vi "Helper Loop.vi"(8 "error in (no error)":errorcluster, 9 "Message Data":variant, 10 "Message":string, 11 "Helper Loop In":refnum<class "Helper Loop.lvclass">) -> (0 "error out":errorcluster, 3 "Helper Loop Out":refnum<class "Helper Loop.lvclass">)   [LabVIEW 2020, in "Helper Loop.lvclass"]
uses:
  Helper Loop.lvclass
  Process/Process.lvclass
  Process/Process.lvclass/Process.ctl
  Process/Public/Lifecycle/Lifecycle State.ctl
  Error Handler Interface/Error Handler Interface.lvclass
  Broadcast Event Helpers/Execution timer.vi
  Logging/Log Error.vi
  Logging/Log Warning.vi
  <vilib>/Utility/error.llb/Clear Errors.vi
  <vilib>/Utility/error.llb/Error Cluster From Error Code.vi
  Broadcast Event Dequeuers/Dequeue Broadcast Message.vi
  Logging/Logging.lvclass
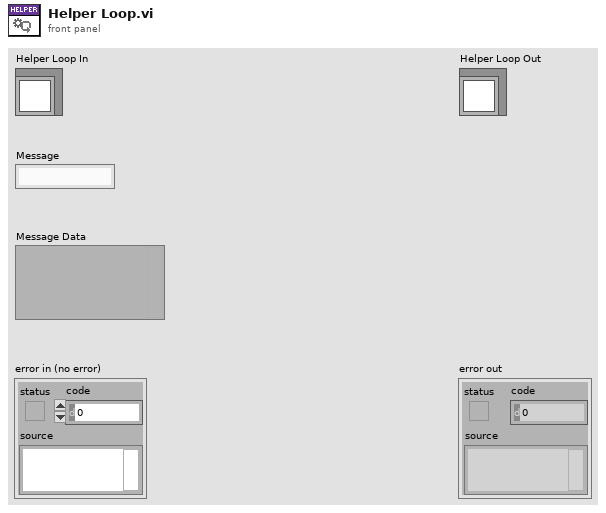
[diagram p1: front panel]
types:
  T1 = typedef "Process.lvclass/Lifecycle State.ctl" = enum16{"Uninitialized", "Initialized", "Started", "Running", "Stopped", "Finished"}
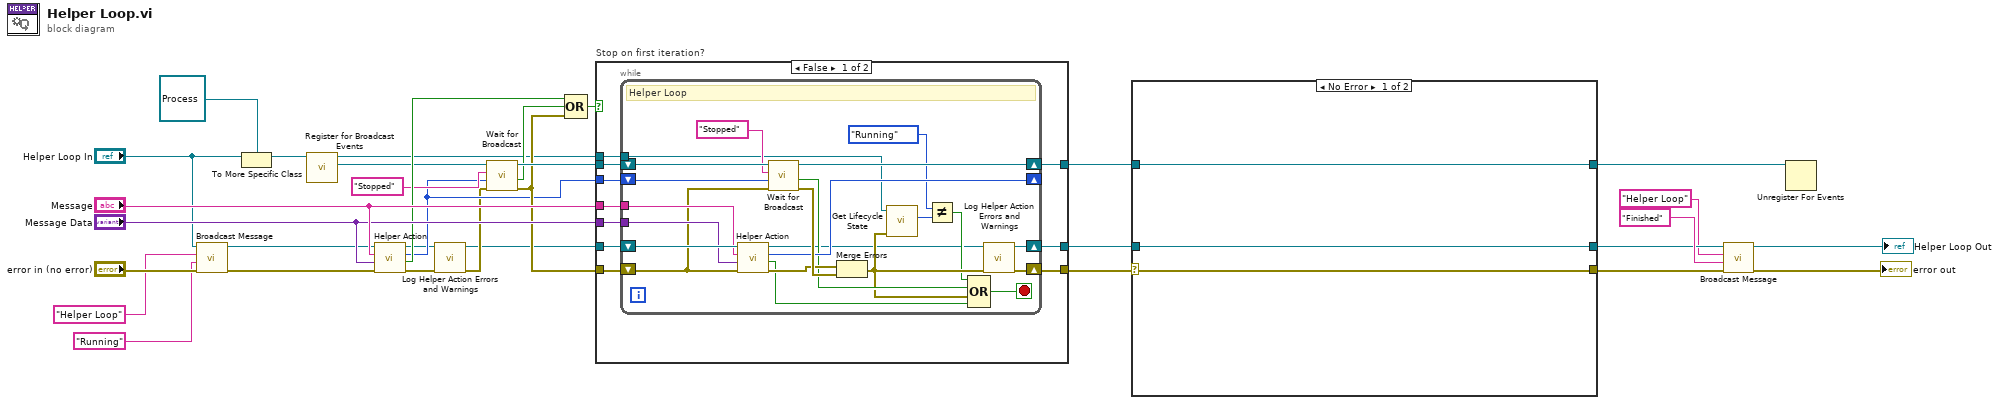
[diagram p0: block diagram]
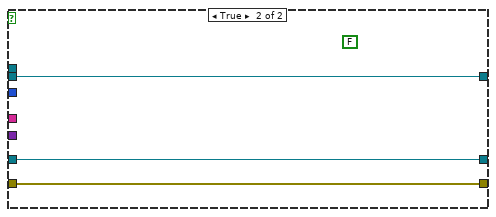
[diagram p2: hidden frame]
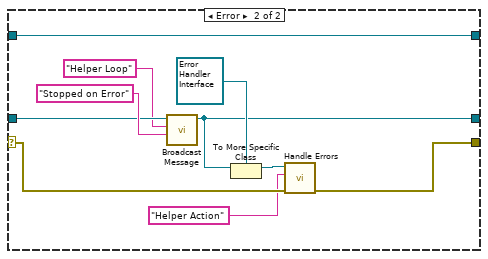
[diagram p3: hidden frame]
diagram:
  n1 = call-dynamic "Broadcast Message.vi"("error in (no error)"="error in (no error)", "Message Data"="Running" ("Message"), "Message"="Helper Loop", "Helper Loop in"="Helper Loop In") -> ("error out"=w8:errorcluster, "Helper Loop out"=w23:refnum<class "Helper Loop.lvclass">)  [unwired: 6 in]
  n2 = To More Specific Class(target class=refnum<class "Process.lvclass"> refnum ("Process.lvclass"), reference="Helper Loop In") -> (specific class reference=w10:refnum<class "Process.lvclass">)  [unwired: 1 in, 1 out]
  n3 = call "Register for Broadcast Events.vi"("Process In"=w10) -> ("Event Registration Refnum Out"=w9:refnum<event-registration>, "Process Out"=w1:refnum<class "Process.lvclass">)  [unwired: 8 in, 1 out]
  n4 = call-dynamic "Helper Action.vi"("error in (no error)"=w8, "Message Data"="Message Data", "Message"="Message", "Helper Loop In"=w23) -> ("error out"=w5:errorcluster, "Exit?"=w24:bool, "Loop Period [ms]"=w6:u32, "Helper Loop Out"=w3:refnum<class "Helper Loop.lvclass">)  [unwired: 4 in]
  n5 = call "Log Helper Action Errors and Warnings.vi"("error in (no error)"=w5, "Helper Loop in"=w3) -> ("error out"=w4:errorcluster, "Helper Loop Out"=w2:refnum<class "Helper Loop.lvclass">)  [unwired: 8 in]
  n6 = call "Wait for Broadcast.vi"("error in (no error)"=w4, "Timeout [ms]"=w6, "Broadcast Message"="Stopped", "Event Registration Refnum in"=w9) -> ("error out"=w20:errorcluster, "Stop Received?"=w13:bool, "Event Registration Refnum out"=w28:refnum<event-registration>)  [unwired: 5 in]
  n7 = Compound Arithmetic op=OR(w24, w13, w20) -> (w25:bool)
  n8 = case "Stop on first iteration?" shown="False" w25 {
    tunnel: [w43 w67] -> w30
    tunnel: [w42 w66] -> w29
    tunnel: [w41 w68] -> w22
    tunnel: w2 -> [w40 w67]
    tunnel: w28 -> [w39 w68]
    tunnel: w20 -> [w38 w66]
    tunnel: "Message" -> [w37 _]
    tunnel: "Message Data" -> [w36 _]
    tunnel: w6 -> [w35 _]
    tunnel: w1 -> [w34 _]
    frame False {
      n9 = while {
        shift-right: [w50] -> w43
        shift-left: w40 -> [w65]
        shift-right: [w51] -> w42
        shift-left: w38 -> [w55]
        tunnel: w37 -> [w62]
        tunnel: w36 -> [w61]
        shift-right: [w57] -> _
        shift-left: w35 -> [w59]
        shift-right: [w56] -> w41
        shift-left: w39 -> [w60]
        tunnel: w34 -> [w49]
        stop <- w64 stop-if-true
        # "Helper Loop"
        n10 = call-dynamic "Helper Action.vi"("error in (no error)"=w55, "Message Data"=w61, "Message"=w62, "Helper Loop In"=w65) -> ("error out"=w58:errorcluster, "Exit?"=w54:bool, "Loop Period [ms]"=w57:u32, "Helper Loop Out"=w44:refnum<class "Helper Loop.lvclass">)  [unwired: 4 in]
        n11 = call "Wait for Broadcast.vi"("error in (no error)"=w55, "Timeout [ms]"=w59, "Broadcast Message"="Stopped", "Event Registration Refnum in"=w60) -> ("error out"=w63:errorcluster, "Stop Received?"=w53:bool, "Event Registration Refnum out"=w56:refnum<event-registration>)  [unwired: 5 in]
        n12 = Merge Errors(w58, w63) -> (w46:errorcluster)
        n13 = call "Get Lifecycle State.vi"("error in (no error)"=w46, "Process In"=w49) -> ("Lifecycle State"=w47:T1)  [unwired: 6 in, 3 out]
        n14 = Not Equal?(x=Lifecycle_State."Running" ("Lifecycle State"), y=w47) -> (x != y?=w45:bool)
        n15 = Compound Arithmetic op=OR(w45, w53, w46, w54) -> (w64:bool)
        n16 = call "Log Helper Action Errors and Warnings.vi"("error in (no error)"=w46, "Helper Loop in"=w44) -> ("error out"=w51:errorcluster, "Helper Loop Out"=w50:refnum<class "Helper Loop.lvclass">)  [unwired: 8 in]
      }
    }
    frame True {
      (unwired) FALSE ("Stop Received?")
    }
  }
  n17 = case shown="No Error" w29 {
    selector: w29 -> [w71 w76]
    tunnel: w30 -> [w69 w80]
    tunnel: [w69 w74] -> w18
    tunnel: [w71 w75] -> w17
    tunnel: w22 -> [w70 w79]
    tunnel: [w70 w79] -> w21
    frame No Error {
    }
    frame Error {
      n18 = call-dynamic "Broadcast Message.vi"("Message Data"="Stopped on Error" ("Description"), "Message"="Helper Loop", "Helper Loop in"=w80) -> ("Helper Loop out"=w74:refnum<class "Helper Loop.lvclass">)  [unwired: 7 in, 1 out]
      n19 = To More Specific Class(target class=refnum<class "Error Handler Interface.lvclass"> refnum ("Error Handler Interface.lvclass"), reference=w74) -> (specific class reference=w77:refnum<class "Error Handler Interface.lvclass">)  [unwired: 1 in, 1 out]
      n20 = call-dynamic "Handle Errors.vi"("error in (no error)"=w76, "Location"="Helper Action" ("format string"), "Error Handler Interface In"=w77) -> ("error out"=w75:errorcluster)  [unwired: 7 in, 1 out]
    }
  }
  n21 = call-dynamic "Broadcast Message.vi"("error in (no error)"=w17, "Message Data"="Finished" ("Description"), "Message"="Helper Loop", "Helper Loop in"=w18) -> ("error out"=→"error out":errorcluster, "Helper Loop out"=→"Helper Loop Out":refnum<class "Helper Loop.lvclass">)  [unwired: 6 in]
  n22 = Unregister For Events(event registration refnum=w21) -> ()  [unwired: 1 in, 1 out]
